vi "TeleOp Default.vi"(10 "Occurrence Refnum":refnum<k4>, 11 "OpMode Index":u64 format="%.0x") -> ()   [LabVIEW 2023]
uses:
  <vilib>/MRC/MrcLib.lvlib
  <vilib>/MRC/Types/WPI_JoystickDeviceEnum.ctl
panel:
  out "RobotMode":u8
  out "Match Time(s)":sgl
  # "Do not rename these\ntwo controls"
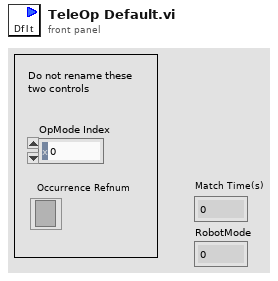
[diagram p1: front panel]
types:
  T1 = typedef "WPI_JoystickDeviceEnum.ctl" = enum16{"USB 0", "USB 1", "USB 2", "USB 3", "USB 4", "USB 5"}
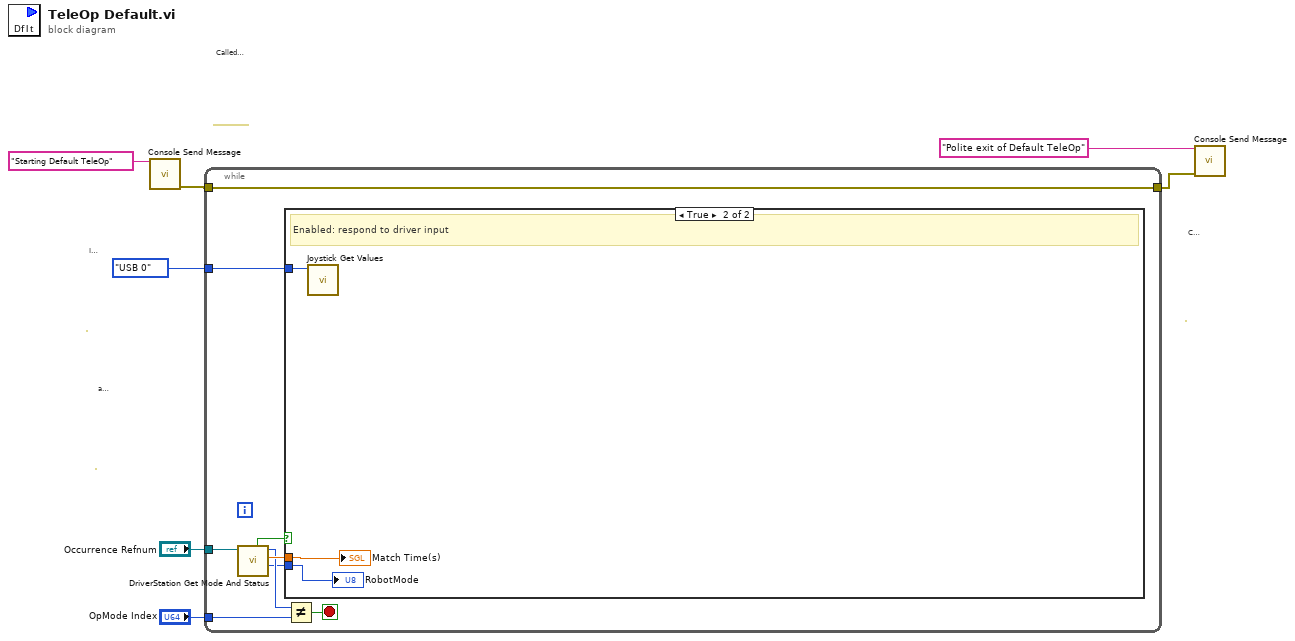
[diagram p0: block diagram]
diagram:
  # "add enabled counter\nstats, etc"
  # "Cleanup I/O"
  # "Called once when teleOp is selected by DS.\nLoop until mode changes carrying out enabled\nor disabled response."
  # "Init I/O and anything\nused during TeleOp"
  n1 = call <vilib>:"Console Send Message.vi"("Message"="Starting Default TeleOp") -> ("error out"=w5:errorcluster)  [unwired: 14 in]
  n2 = while {
    tunnel: "OpMode Index" -> [w14]
    tunnel: [w10] -> w3
    tunnel: w5 -> [w10]
    tunnel: "Occurrence Refnum" -> [w9]
    tunnel: WPI_JoystickDeviceEnum."USB 0" ("Joystick") -> [w8]
    stop <- w13 stop-if-true
    n3 = call <vilib>:"DriverStation Get Mode And Status.vi"("Occurrence Refnum"=w9) -> ("RobotMode"=w11:u8, "Match Time(s)"=w16:sgl, "currentOpMode"=w12:u64, "Enabled"=w15:bool)  [unwired: 5 in, 2 out]
    n4 = case shown="True" w15 {
      tunnel: w16 -> [_ w19]
      tunnel: w11 -> [_ w18]
      tunnel: w8 -> [_ w17]
      frame False {
        # "Disabled: update dashboard, possibly update state and setpoints for safer enable"
      }
      frame True {
        # "Enabled: respond to driver input"
        n5 = call <vilib>:"Joystick Get Values.vi"("Joystick"=w17) -> ()  [unwired: 5 in, 6 out]
        "Match Time(s)" <- w19
        "RobotMode" <- w18
      }
    }
    n6 = Not Equal?(x=w12, y=w14) -> (x != y?=w13:bool)
  }
  n7 = call <vilib>:"Console Send Message.vi"("Message"="Polite exit of Default TeleOp", "error in (no error)"=w3) -> ()  [unwired: 13 in, 1 out]
